vi "[ex ce] Calc FFT.vi"() -> ()   [LabVIEW 2021]
doc: "<B>Signal processing example</B>\n\nA script in this example generates a waveform array and calculates some parameters of it using FFT. Then it restores the waveform with the help of Inverse FFT.\n\nResults of computation are displaied in graphs on the Front Panel. \n\n<B>Remark</B>\nSome functions in this example use VIs of Advanced Analysis Package. The example doesn't work properly if you don't have these VIs.\n\n::: CalcExpress Toolkit :::\nCopyright (c) 2000-2026 Konstantin Shifershteyn. All rights reserved."
panel:
  in  "Restored Signal - Variable Name":string="Restored"
  in  "Initial Signal - Variable Name":string="Signal"
  out "WaveForm":dbl[][](graph)
  in  "FFT phase - Variable Name":string="fft_ph"
  out "spectrum phase":dbl[](graph)
  in  "FFT magnitude - Variable Name":string="fft_mag"
  out "spectrum":dbl[](graph)
  in  "stop":bool
  in  "Expression":string="dbl(\"Phase\",0);\na1dbl(\"Signal\");\nFs = 1000; // Sampling frequency\nNs = 100;  // Number of samples\nF  = 39;   // Waveform frequency\n\n/*\nCreate a waveform and place it to Signal variable.\nThe Phase variable is to be reused when the script is executed next time.\n*/\nPhase = SquareWave(Signal,Ns,F/Fs,6, Phase, 40);\n\n/* Compute FFT of Signal */\nfft = FFT(Signal);\n\n/* Compute magnitude & phase of FFT */\nsz = size(fft)/2;   // half of array size\nfft_mag = abs( fft[0:sz-1] );\nfft_ph  = arg( fft[0:sz-1] );\n\n/*\n1. restore signal using Inverse FFT: iFFT(fft)\n2. reduce its magnitude: /2\n3. reverse the signal array\n*/\nRestored = reverse( iFFT(fft)/2);\n"
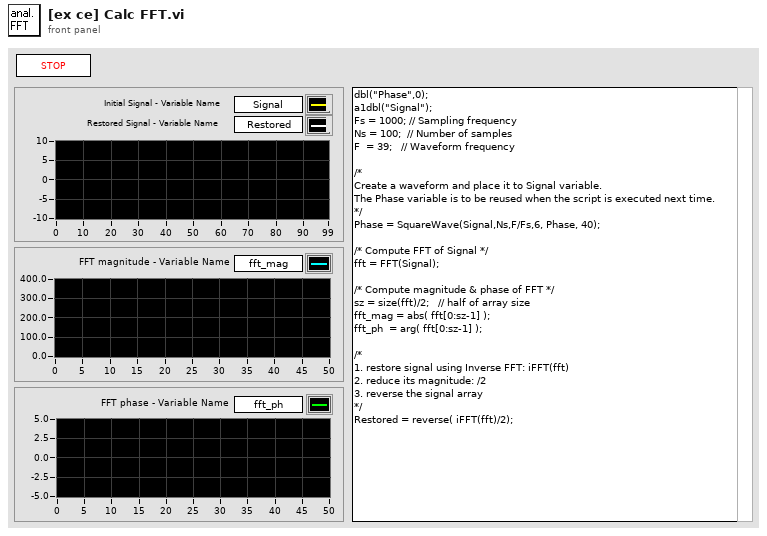
[diagram p1: front panel]
types:
  T1 = enum32{"nothing", "reset", "assign name", "get name", "get handle"}
  T2 = typedef "VarMan Variable Context Handle.ctl" = i32
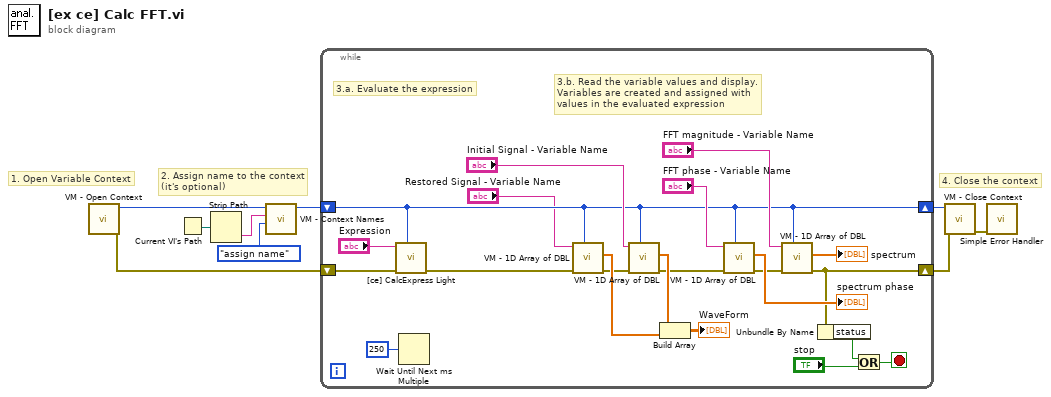
[diagram p0: block diagram]
diagram:
  # "4. Close the context"
  # "1. Open Variable Context"
  # "2. Assign name to the context\n(it's optional)"
  n1 = call "VM - Open Context.vi"() -> ("error out"=w9:errorcluster, "VC Handle out"=w3:T2)  [unwired: 9 in, 1 out]
  n2 = Current VI's Path() -> (path=w5:path)
  n3 = Strip Path(path=w5) -> (name=w4:string)  [unwired: 1 out]
  n4 = call "VM - Context Names.vi"("action"=T1."assign name", "VC Name"=w4, "VC Handle"=w3) -> ("VC Handle out"=w2:T2)  [unwired: 3 in, 3 out]
  n5 = while {
    shift-left: w9 -> [w20]
    shift-right: [w15] -> w8
    shift-right: [w11] -> w1
    shift-left: w2 -> [w11]
    stop <- w12 stop-if-true
    # "3.b. Read the variable values and display.\nVariables are created and assigned with\nvalues in the evaluated expression"
    # "3.a. Evaluate the expression"
    n6 = call "[ce] CalcExpress Light.vi"("VC Handle"=w11, "error in"=w20, "expression"="Expression") -> ("error out"=w19:errorcluster)  [unwired: 6 in, 2 out]
    n7 = Wait Until Next ms Multiple(millisecond multiple=u32 250 ("milliseconds to wait")) -> ()  [unwired: 1 out]
    n8 = call "VM - 1D Array of DBL.vi"("VC Handle"=w11, "error in"=w19, "name_spec"="Restored Signal - Variable Name") -> ("error out"=w18:errorcluster, "value out"=w23:dbl[])  [unwired: 3 in, 4 out]
    n9 = call "VM - 1D Array of DBL.vi"("VC Handle"=w11, "error in"=w18, "name_spec"="Initial Signal - Variable Name") -> ("error out"=w17:errorcluster, "value out"=w24:dbl[])  [unwired: 3 in, 4 out]
    n10 = Build Array(w24, w23) -> (→"WaveForm":dbl[][])
    n11 = call "VM - 1D Array of DBL.vi"("VC Handle"=w11, "error in"=w17, "name_spec"="FFT phase - Variable Name") -> ("error out"=w16:errorcluster, "value out"=→"spectrum phase":dbl[])  [unwired: 3 in, 4 out]
    n12 = call "VM - 1D Array of DBL.vi"("VC Handle"=w11, "error in"=w16, "name_spec"="FFT magnitude - Variable Name") -> ("error out"=w15:errorcluster, "value out"=→"spectrum":dbl[])  [unwired: 3 in, 4 out]
    n13 = Unbundle By Name(w15) -> ("status"=w14:bool)
    n14 = Or(x=w14, y="stop") -> (x .or. y?=w12:bool)
  }
  n15 = call "VM - Close Context.vi"("error in"=w8, "VC Handle"=w1) -> ("error out"=w7:errorcluster)  [unwired: 8 in, 1 out]
  n16 = call <vilib>:"Simple Error Handler.vi"("error in (no error)"=w7) -> ()  [unwired: 4 in, 5 out]
